vi "PicoScope4000aAdvancedTriggerSettings.vi"(0 "handle in":i16, 5 "error in":errorcluster, 6 "Trigger Conditions":T4 {"Channel H" items=["Don't Care", "True", "False"]; "Channel G" items=["Don't Care", "True", "False"]; "Channel F" items=["Don't Care", "True", "False"]; "Channel E" items=["Don't Care", "True", "False"]; "PWQ" items=["Don't Care", "True", "False"]; "Aux" items=["Don't Care", "True", "False"]; "Ext" items=["Don't Care", "True", "False"]; "Channel D" items=["Don't Care", "True", "False"]; "Channel C" items=["Don't Care", "True", "False"]; "Channel B" items=["Don't Care", "True", "False"]; "Channel A" items=["Don't Care", "True", "False"]; "Condition Logic" items=["AND", "OR", "XOR"]}, 8 "Channel Trigger Properties":T2 {"Channel H Trigger Properties"."Direction" items=["Above / Inside", "Below / Outside", "Rising / Enter", "Falling / Exit", "Rising or Falling / Enter or Exit", "Above Lower", "Below Lower", "Rising Lower", "Falling Lower", "Positive Runt", "Negative Runt"]; "Channel H Trigger Properties"."Threshold Mode" items=["Level", "Window"]; "Channel G Trigger Properties"."Direction" items=["Above / Inside", "Below / Outside", "Rising / Enter", "Falling / Exit", "Rising or Falling / Enter or Exit", "Above Lower", "Below Lower", "Rising Lower", "Falling Lower", "Positive Runt", "Negative Runt"]; "Channel G Trigger Properties"."Threshold Mode" items=["Level", "Window"]; "Channel F Trigger Properties"."Direction" items=["Above / Inside", "Below / Outside", "Rising / Enter", "Falling / Exit", "Rising or Falling / Enter or Exit", "Above Lower", "Below Lower", "Rising Lower", "Falling Lower", "Positive Runt", "Negative Runt"]; "Channel F Trigger Properties"."Threshold Mode" items=["Level", "Window"]; "Channel E Trigger Properties"."Direction" items=["Above / Inside", "Below / Outside", "Rising / Enter", "Falling / Exit", "Rising or Falling / Enter or Exit", "Above Lower", "Below Lower", "Rising Lower", "Falling Lower", "Positive Runt", "Negative Runt"]; "Channel E Trigger Properties"."Threshold Mode" items=["Level", "Window"]; "Channel D Trigger Properties"."Direction" items=["Above / Inside", "Below / Outside", "Rising / Enter", "Falling / Exit", "Rising or Falling / Enter or Exit", "Above Lower", "Below Lower", "Rising Lower", "Falling Lower", "Positive Runt", "Negative Runt"]; "Channel D Trigger Properties"."Threshold Mode" items=["Level", "Window"]; "Channel C Trigger Properties"."Direction" items=["Above / Inside", "Below / Outside", "Rising / Enter", "Falling / Exit", "Rising or Falling / Enter or Exit", "Above Lower", "Below Lower", "Rising Lower", "Falling Lower", "Positive Runt", "Negative Runt"]; "Channel C Trigger Properties"."Threshold Mode" items=["Level", "Window"]; "Channel B Trigger Properties"."Direction" items=["Above / Inside", "Below / Outside", "Rising / Enter", "Falling / Exit", "Rising or Falling / Enter or Exit", "Above Lower", "Below Lower", "Rising Lower", "Falling Lower", "Positive Runt", "Negative Runt"]; "Channel B Trigger Properties"."Threshold Mode" items=["Level", "Window"]; "Channel A Trigger Properties"."Direction" items=["Above / Inside", "Below / Outside", "Rising / Enter", "Falling / Exit", "Rising or Falling / Enter or Exit", "Above Lower", "Below Lower", "Rising Lower", "Falling Lower", "Positive Runt", "Negative Runt"]; "Channel A Trigger Properties"."Threshold Mode" items=["Level", "Window"]}, 9 "Addition Trigger Properties":T3 {"Aux. Trigger Properties (DO NOT USE)"."Direction" items=["Above / Inside", "Below / Outside", "Rising / Enter", "Falling / Exit", "Rising or Falling / Enter or Exit", "Above Lower", "Below Lower", "Rising Lower", "Falling Lower", "Positive Runt", "Negative Runt"]; "Aux. Trigger Properties (DO NOT USE)"."Threshold Mode" items=["Level", "Window"]; "Ext. Trigger Properties"."Direction" items=["Above / Inside", "Below / Outside", "Rising / Enter", "Falling / Exit", "Rising or Falling / Enter or Exit", "Above Lower", "Below Lower", "Rising Lower", "Falling Lower", "Positive Runt", "Negative Runt"]; "Ext. Trigger Properties"."Threshold Mode" items=["Level", "Window"]}, 10 "Auto Trigger (ms)":i32, 11 "Pulse Width Qualifier Conditions":T1 {"Channel H" items=["Don't Care", "True", "False"]; "Channel G" items=["Don't Care", "True", "False"]; "Channel F" items=["Don't Care", "True", "False"]; "Channel E" items=["Don't Care", "True", "False"]; "Aux" items=["Don't Care", "True", "False"]; "Ext" items=["Don't Care", "True", "False"]; "Channel D" items=["Don't Care", "True", "False"]; "Channel C" items=["Don't Care", "True", "False"]; "Channel B" items=["Don't Care", "True", "False"]; "Channel A" items=["Don't Care", "True", "False"]; "Condition Logic" items=["AND", "OR", "XOR"]}, 12 "Trigger Delay":u32, 13 "Pulse Width Qualifier Settings":T5 {"Pulse Width Type" items=["None", "Less Than", "Greater Than", "In Range", "Out of Range"]; "Direction" items=["Rising", "Falling", "Rising Lower", "Above", "Below", "Rising or Falling", "Falling Lower", "Below Lower", "Above Lower"]}) -> (14 "handle out":i16, 19 "error out":errorcluster)   [LabVIEW 2009]
doc: "This VI is an interface for the advanced trigger features of the oscilloscope.\nA simple trigger can be set using PicoScopeXXXXSettings.vi, in which case it is not necessary to use this VI."
uses:
  Program Files/Pico Technology/SDK/lib/ps4000a.dll
panel:
  in  "PWQ Info Action XOR":bool
  in  "PWQ Info Action OR":bool
  in  "SetTrigger Info Action XOR":bool
  out "XOR Debug Array":u32[][](array[numeric])
  in  "SetTrigger Info Action OR":bool
  # "For Condition Logic Suggested settings;\nFor AND, XOR logic-(parallel triggers)\nUse level-type triggers (Level or Inside/outside Window Triggers)\n\nFor OR logic- (single channel)\nUse edge types (e.g. rising, falling, entering window)"
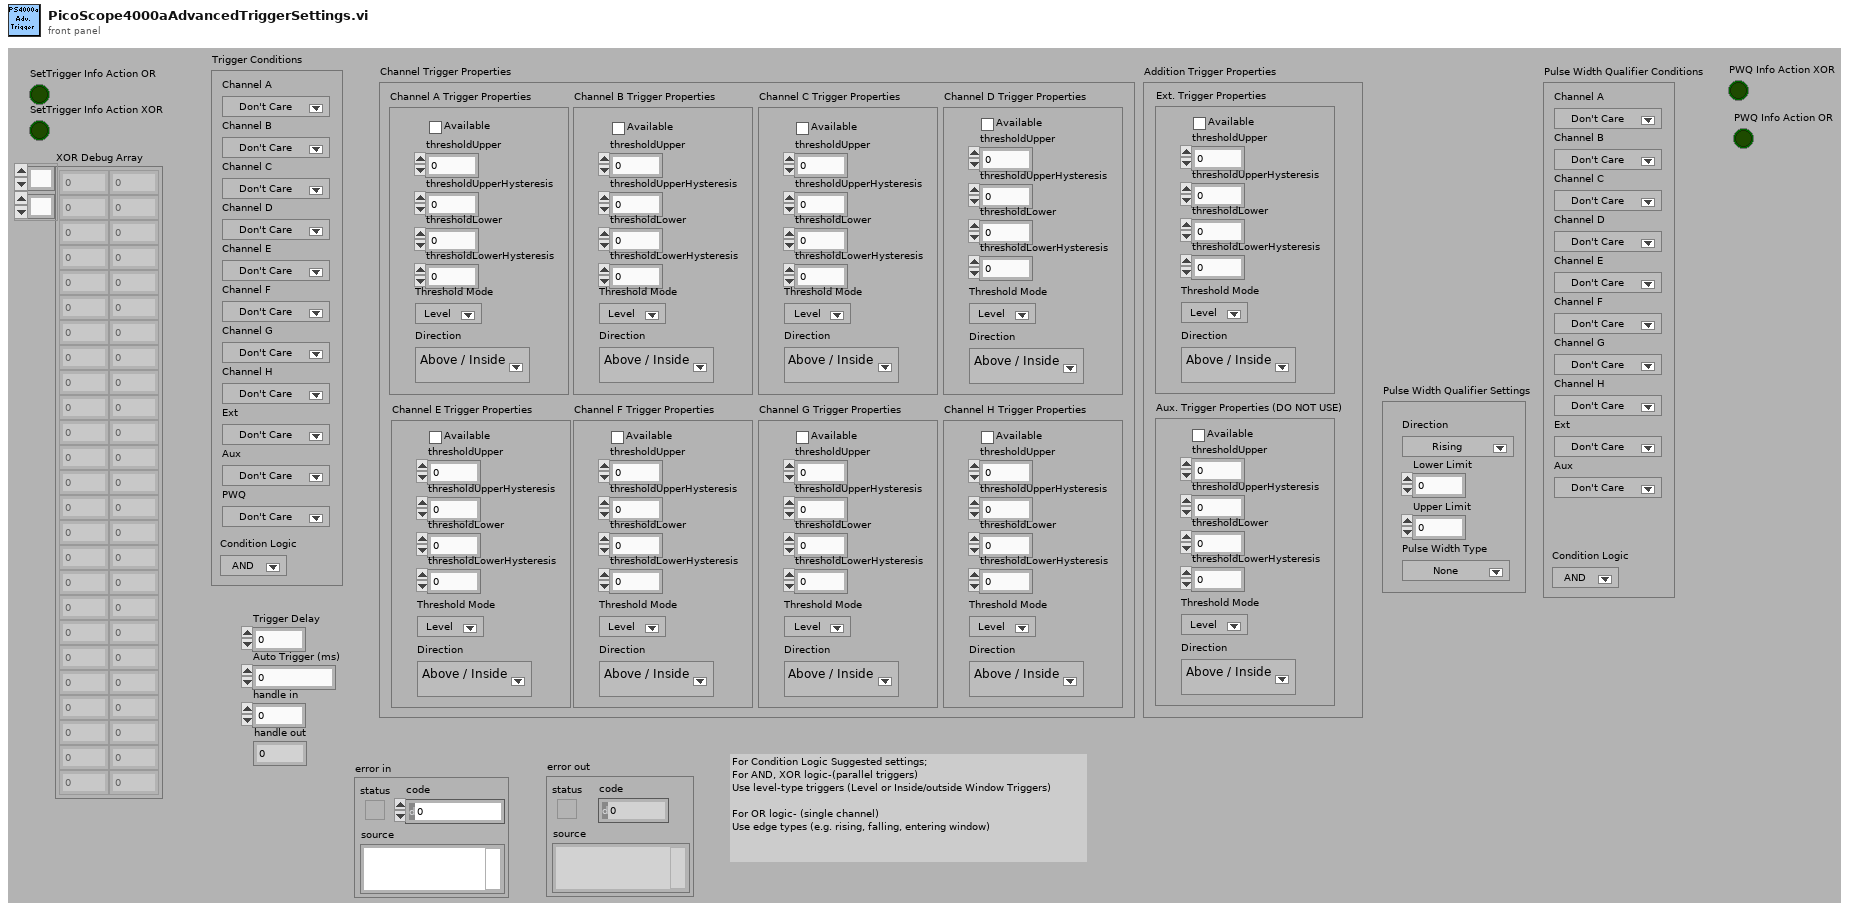
[diagram p1: front panel]
types:
  T1 = cluster{"Channel A":u16, "Channel B":u16, "Channel C":u16, "Channel D":u16, "Channel E":u16, "Channel F":u16, "Channel G":u16, "Channel H":u16, "Ext":u16, "Aux":u16, "Condition Logic":u16}
  T2 = cluster{"Channel A Trigger Properties":cluster{"thresholdUpper":i16, "thresholdUpperHysteresis":u16, "thresholdLower":i16, "thresholdLowerHysteresis":u16, "Threshold Mode":i32, "Direction":i32, "Available":bool}, "Channel B Trigger Properties":cluster{"thresholdUpper":i16, "thresholdUpperHysteresis":u16, "thresholdLower":i16, "thresholdLowerHysteresis":u16, "Threshold Mode":i32, "Direction":i32, "Available":bool}, "Channel C Trigger Properties":cluster{"thresholdUpper":i16, "thresholdUpperHysteresis":u16, "thresholdLower":i16, "thresholdLowerHysteresis":u16, "Threshold Mode":i32, "Direction":i32, "Available":bool}, "Channel D Trigger Properties":cluster{"thresholdUpper":i16, "thresholdUpperHysteresis":u16, "thresholdLower":i16, "thresholdLowerHysteresis":u16, "Threshold Mode":i32, "Direction":i32, "Available":bool}, "Channel E Trigger Properties":cluster{"thresholdUpper":i16, "thresholdUpperHysteresis":u16, "thresholdLower":i16, "thresholdLowerHysteresis":u16, "Threshold Mode":i32, "Direction":i32, "Available":bool}, "Channel F Trigger Properties":cluster{"thresholdUpper":i16, "thresholdUpperHysteresis":u16, "thresholdLower":i16, "thresholdLowerHysteresis":u16, "Threshold Mode":i32, "Direction":i32, "Available":bool}, "Channel G Trigger Properties":cluster{"thresholdUpper":i16, "thresholdUpperHysteresis":u16, "thresholdLower":i16, "thresholdLowerHysteresis":u16, "Threshold Mode":i32, "Direction":i32, "Available":bool}, "Channel H Trigger Properties":cluster{"thresholdUpper":i16, "thresholdUpperHysteresis":u16, "thresholdLower":i16, "thresholdLowerHysteresis":u16, "Threshold Mode":i32, "Direction":i32, "Available":bool}}
  T3 = cluster{"Ext. Trigger Properties":cluster{"thresholdUpper":i16, "thresholdUpperHysteresis":u16, "thresholdLower":i16, "thresholdLowerHysteresis":u16, "Threshold Mode":i32, "Direction":i32, "Available":bool}, "Aux. Trigger Properties (DO NOT USE)":cluster{"thresholdUpper":i16, "thresholdUpperHysteresis":u16, "thresholdLower":i16, "thresholdLowerHysteresis":u16, "Threshold Mode":i32, "Direction":i32, "Available":bool}}
  T4 = cluster{"Channel A":u16, "Channel B":u16, "Channel C":u16, "Channel D":u16, "Channel E":u16, "Channel F":u16, "Channel G":u16, "Channel H":u16, "Ext":u16, "Aux":u16, "PWQ":u16, "Condition Logic":u16}
  T5 = cluster{"Direction":u32, "Lower Limit":u32, "Upper Limit":u32, "Pulse Width Type":u32}
  T6 = cluster{"status":bool, "code":u32, "source":string}
  T7 = cluster{"status":bool, "code":u32, "source":string}[]
  T8 = cluster{"thresholdUpper":i16, "thresholdUpperHysteresis":u16, "thresholdLower":i16, "thresholdLowerHysteresis":u16, "Threshold Mode":i32, "Direction":i32, "Available":bool}[]
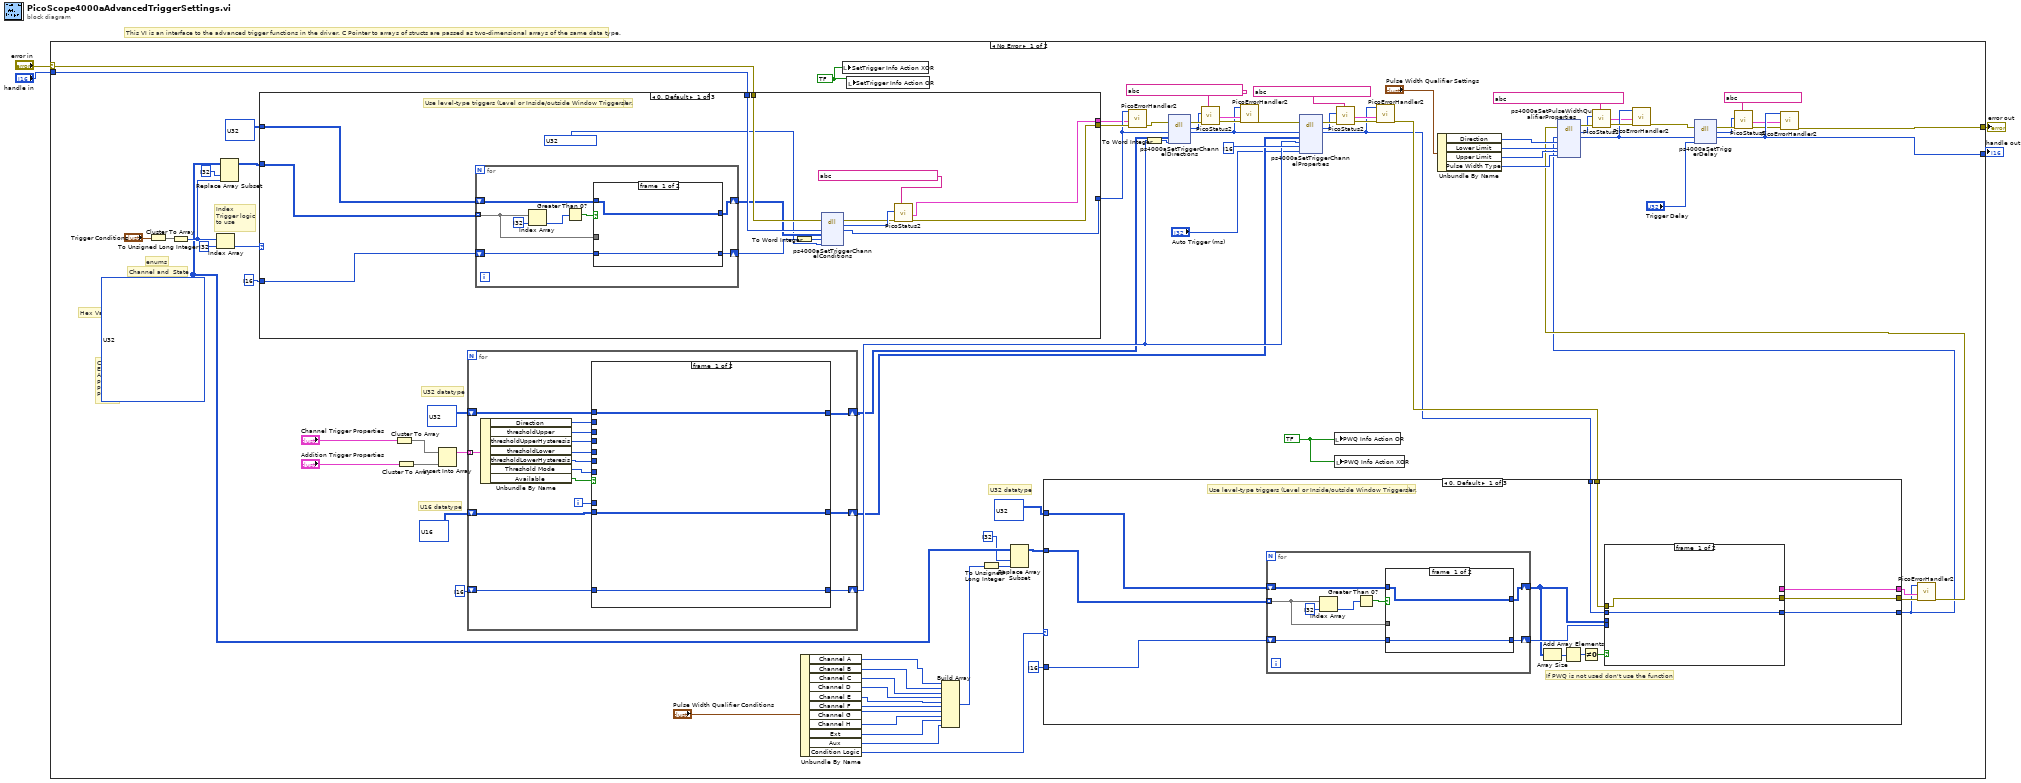
[diagram p0: block diagram]
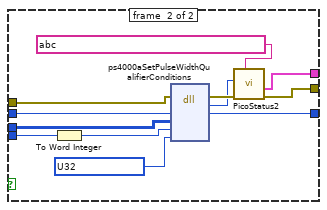
[diagram p2: hidden frame]
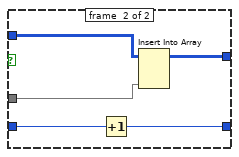
[diagram p3: hidden frame]
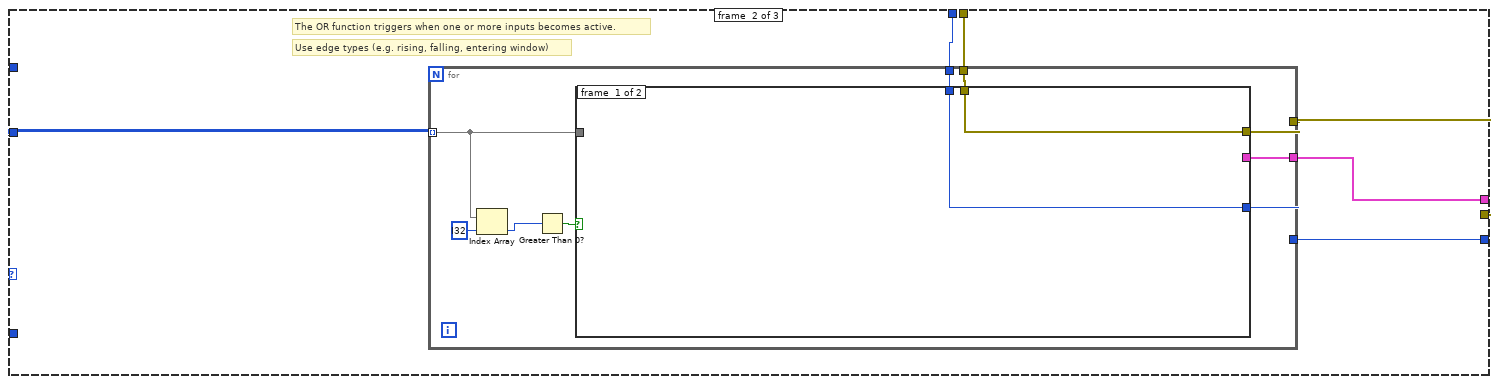
[diagram p4: hidden frame]
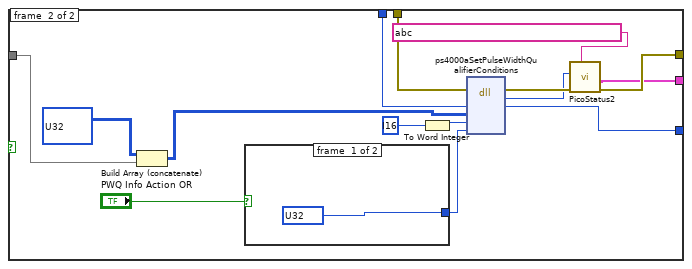
[diagram p5: hidden frame]
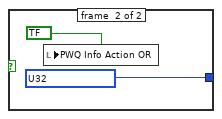
[diagram p6: hidden frame]
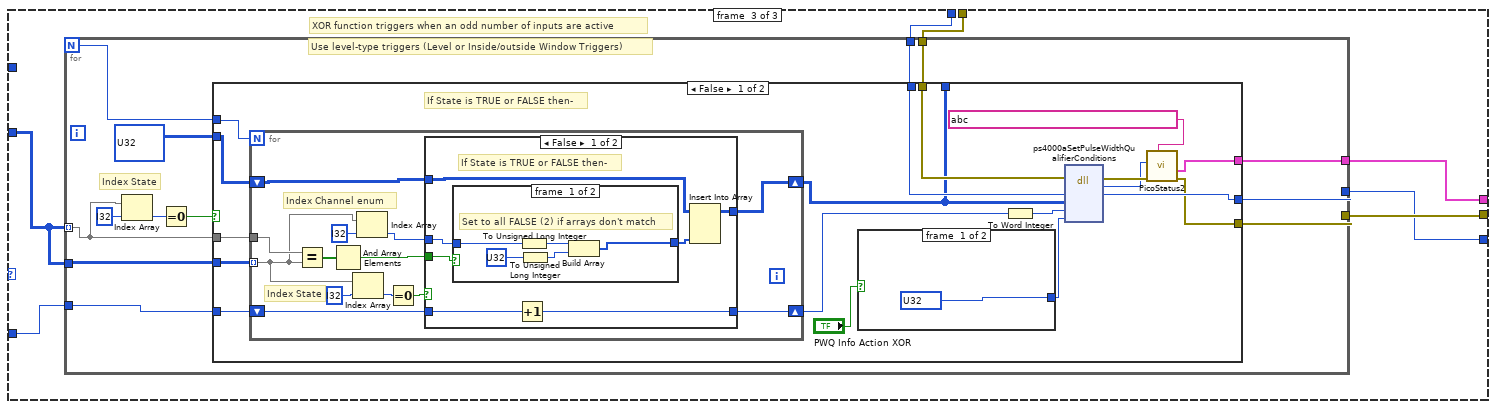
[diagram p7: hidden frame]
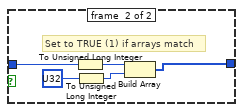
[diagram p8: hidden frame]
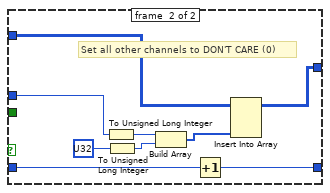
[diagram p9: hidden frame]
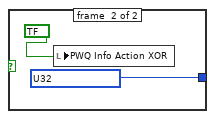
[diagram p10: hidden frame]
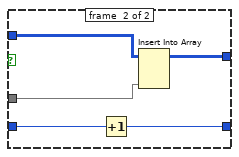
[diagram p12: hidden frame]
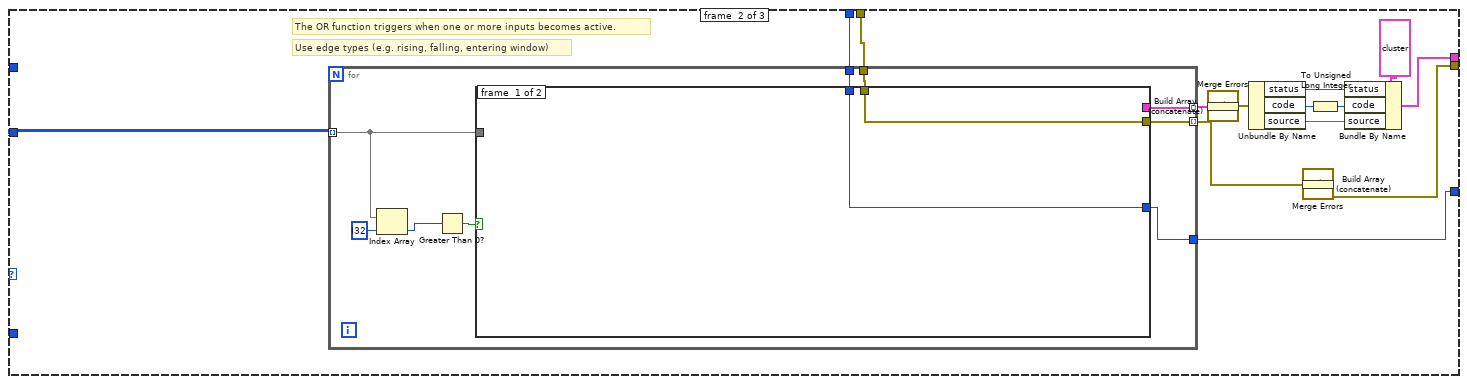
[diagram p13: hidden frame]
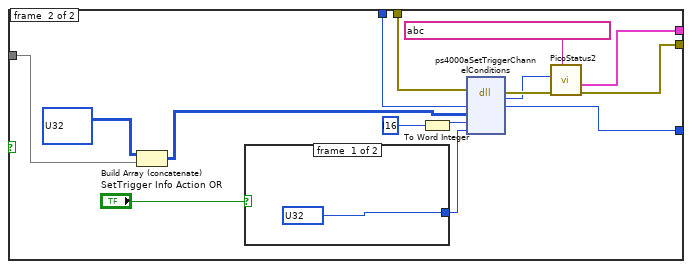
[diagram p14: hidden frame]
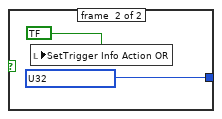
[diagram p15: hidden frame]
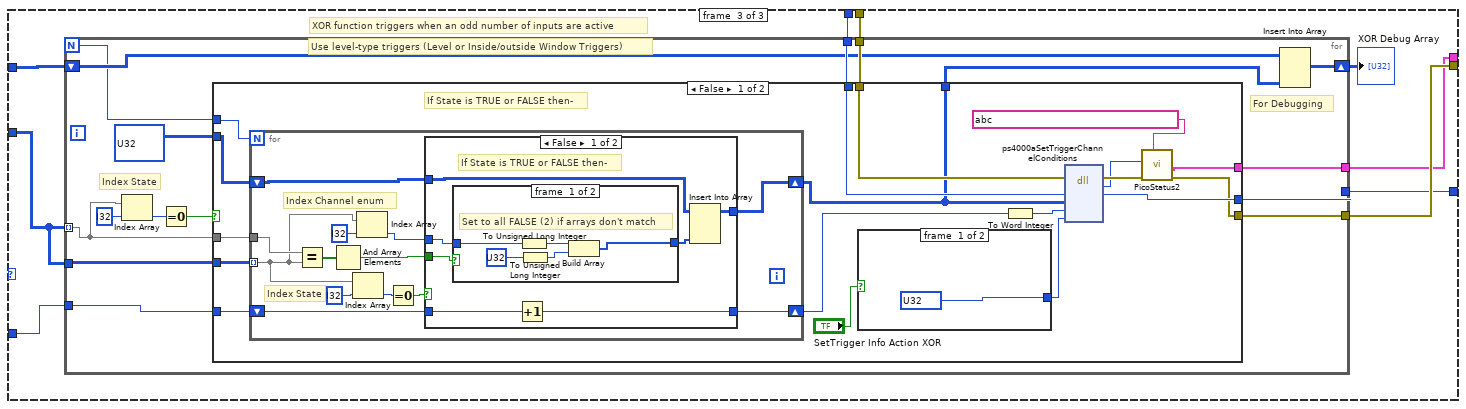
[diagram p16: hidden frame]
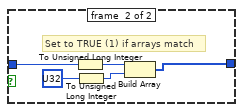
[diagram p17: hidden frame]
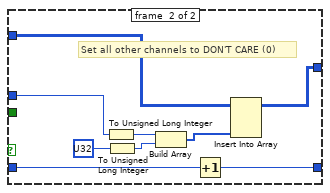
[diagram p18: hidden frame]
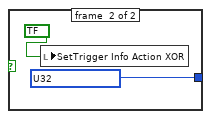
[diagram p19: hidden frame]
diagram:
  # "This VI is an interface to the advanced trigger functions in the driver. C Pointer to arrays of structs are passed as two-dimensional arrays of the same data type."
  n1 = case shown="No Error" "error in" {
    selector: "error in" -> [w59 w459]
    tunnel: "handle in" -> [w58 w460]
    tunnel: [w74 w460] -> w2
    tunnel: [w75 w459] -> w1
    frame #0 {
      w33 = bool ? ("PWQ Info Action XOR")
      w65 = bool ? ("Boolean")
      w48 = u32[][] ?
      # "U32 datatype"
      # "Index\nTrigger logic\nto use"
      # "enums"
      # "Ch H\nExt\nAux\nPWQ\nPort0\nPort1"
      # "Channel and  State"
      # "Hex Values"
      # "U16 datatype"
      # "U32 datatype"
      n2 = Cluster To Array(cluster="Trigger Conditions") -> (array=w82:u16[])
      n3 = To Unsigned Long Integer(number=w82) -> (unsigned 32bit integer=w77:u32[])
      n4 = Index Array(array=w77, index=i32 ?) -> (element=w64:u32)
      n5 = Replace Array Subset(array=w48, new element=w77, index (col)=i32 ? ("disabled index (col)")) -> (w63:u32[][])  [unwired: 1 in]
      n6 = case shown="0, Default" w64 {
        tunnel: u32[][] ? -> [w267 _ w332]
        tunnel: i16 ? -> [w266 _ w329]
        tunnel: w59 -> [w263 w298 w336]
        tunnel: w58 -> [w262 w297 w335]
        tunnel: [w253 w293 w334] -> w61
        tunnel: [w259 w296 w333] -> w60
        tunnel: w63 -> [w258 w295 w330]
        tunnel: [w254 w287 w328] -> w9
        frame #0 {
          w260 = u32 ? items=["CLEAR + ADD", "CLEAR", "ADD"] ("Condition Action")
          # "AND function requires both inputs to be active before it will trigger."
          # "Use level-type triggers (Level or Inside/outside Window Triggers)"
          n7 = for {
            shift-right: [w274] -> w264
            shift-left: w266 -> [w273]
            shift-right: [w272] -> w261
            shift-left: w267 -> [w275]
            tunnel: w258 -> [w270] mode=indexing
            n8 = Index Array(array=w270, index=i32 ?) -> (element=w269:u32)
            n9 = Greater Than 0?(x=w269) -> (x > 0?=w271:bool)
            n10 = case shown="True" w271 {
              tunnel: w275 -> [w277 w282]
              tunnel: [w277 w281] -> w272
              tunnel: [w276 w280] -> w274
              tunnel: w273 -> [w276 w279]
              tunnel: w270 -> [_ w278]
              frame #0 {
              }
              frame #1 {
                n11 = Increment(x=w279) -> (x+1=w280:i16)
                n12 = Insert Into Array(array=w282, new element=w278) -> (w281:u32[][])  [unwired: 2 in]
              }
            }
          }
          n13 = To Word Integer(number=w264) -> (16bit integer=w265:i16)
          n14 = dll-call lib="/Program Files/Pico Technology/SDK/lib/ps4000a.dll" fn="ps4000aSetTriggerChannelConditions" ("ps3000.dll:_ps3000_open_unit@0")(error in=w263, "handle"=w262, "conditions"=w261, "nConditions"=w265, "info"=w260) -> (error out=w255:errorcluster, "PICO_STATUS"=w256:u32, "handle"=w259:i16)  [unwired: 5 in, 1 out]
          n15 = call "PicoStatus2.vi"("PICO source"=string ? ("source"), "Error in"=w255, "PICO STATUS"=w256) -> ("error out"=w253:errorcluster, "PICO_STATUS out"=w254:T6)  [unwired: 5 in]
        }
        frame #1 {
          # "Use edge types (e.g. rising, falling, entering window)"
          # "The OR function triggers when one or more inputs becomes active."
          n16 = for {
            tunnel: w298 -> [w307]
            tunnel: w297 -> [w306]
            tunnel: [w305] -> w294 mode=indexing
            tunnel: [w304] -> w296
            tunnel: w295 -> [w302] mode=indexing
            tunnel: [w299] -> w286 mode=indexing
            n17 = Index Array(array=w302, index=i32 ?) -> (element=w301:u32)
            n18 = Greater Than 0?(x=w301) -> (x > 0?=w300:bool)
            n19 = case shown="True" w300 {
              tunnel: w307 -> [w308 w323]
              tunnel: w306 -> [w309 w322]
              tunnel: [w308 w312] -> w305
              tunnel: [w309 w320] -> w304
              tunnel: w302 -> [_ w315]
              tunnel: [_ w310] -> w299
              frame #0 {
              }
              frame #1 {
                n20 = Build Array (concatenate)(u32[][] ?, w315) -> (w317:u32[][])
                n21 = case shown="True" "SetTrigger Info Action OR" {
                  tunnel: [w325 w327] -> w321
                  frame #0 {
                    w325 = u32 ? items=["CLEAR", "ADD", "CLEAR + ADD"] ("Condition Action")
                  }
                  frame #1 {
                    w327 = u32 ? items=["CLEAR", "ADD", "CLEAR + ADD"] ("Condition Action")
                    n22 = local write "SetTrigger Info Action OR"(bool ? ("Boolean")) -> ()
                  }
                }
                n23 = To Word Integer(number=i16 ?) -> (16bit integer=w324:i16)
                n24 = dll-call lib="/Program Files/Pico Technology/SDK/lib/ps4000a.dll" fn="ps4000aSetTriggerChannelConditions" ("ps3000.dll:_ps3000_open_unit@0")(error in=w323, "handle"=w322, "conditions"=w317, "nConditions"=w324, "info"=w321) -> (error out=w314:errorcluster, "PICO_STATUS"=w311:u32, "handle"=w320:i16)  [unwired: 5 in, 1 out]
                n25 = call "PicoStatus2.vi"("PICO source"=string ? ("source"), "Error in"=w314, "PICO STATUS"=w311) -> ("error out"=w312:errorcluster, "PICO_STATUS out"=w310:T6)  [unwired: 5 in]
              }
            }
          }
          n26 = Build Array (concatenate)(w286) -> (w284:T7)
          n27 = call <vilib>:"Merge Errors.vi"("error array in"=w284) -> ("error out"=w285:errorcluster)  [unwired: 6 in]
          n28 = Unbundle By Name(w285) -> ("status"=w289:bool, "code"=w292:i32, "source"=w290:string)
          n29 = Build Array (concatenate)(w294) -> (w283:errorcluster[])
          n30 = call <vilib>:"Merge Errors.vi"("error array in"=w283) -> ("error out"=w293:errorcluster)  [unwired: 6 in]
          n31 = To Unsigned Long Integer(number=w292) -> (unsigned 32bit integer=w291:u32)
          n32 = Bundle By Name(cluster=T6 ? ("PICO_STATUS in"), "status"=w289, "code"=w291, "source"=w290) -> (w287:T6)
        }
        frame #2 {
          # "Use level-type triggers (Level or Inside/outside Window Triggers)"
          # "XOR function triggers when an odd number of inputs are active"
          n33 = for {
            N -> [w345]
            tunnel: w336 -> [w352]
            tunnel: w335 -> [w351]
            tunnel: [w350] -> w334
            tunnel: [w349] -> w333
            shift-right: [w347] -> w331
            shift-left: w332 -> [w348]
            tunnel: w330 -> [w339] mode=indexing
            tunnel: w330 -> [w342]
            tunnel: w329 -> [w343]
            tunnel: [w337] -> w328
            # "Index State"
            # "For Debugging"
            n34 = Index Array(array=w339, index=i32 ?) -> (element=w340:u32)
            n35 = Equal To 0?(x=w340) -> (x = 0?=w338:bool)
            n36 = case shown="False" w338 {
              tunnel: w352 -> [w370 w413]
              tunnel: w351 -> [w369 w414]
              tunnel: [w354 w413] -> w350
              tunnel: [w368 w414] -> w349
              tunnel: [w366 w415] -> w346
              tunnel: w345 -> [w365 _]
              tunnel: u32[][] ? -> [w364 w415]
              tunnel: w343 -> [w363 _]
              tunnel: w342 -> [w362 _]
              tunnel: w339 -> [w361 _]
              tunnel: [w353 _] -> w337
              frame #0 {
                # "If State is TRUE or FALSE then-"
                n37 = for {
                  N: w365 -> [_]
                  shift-right: [w382] -> w367
                  shift-left: w363 -> [w383]
                  shift-right: [w371] -> w366
                  shift-left: w364 -> [w372]
                  tunnel: w361 -> [w379]
                  tunnel: w362 -> [w375] mode=indexing
                  # "Index State"
                  # "Index Channel enum"
                  n38 = Equal?(x=w379, y=w375) -> (x = y?=w373:bool[])
                  n39 = And Array Elements(Boolean array=w373) -> (logical AND=w378:bool)
                  n40 = Index Array(array=w375, index=i32 ?) -> (element=w376:u32)
                  n41 = Index Array(array=w375, index=i32 ?) -> (element=w380:u32)
                  n42 = Equal To 0?(x=w376) -> (x = 0?=w374:bool)
                  n43 = case shown="False" w374 {
                    tunnel: w383 -> [w390 w401]
                    tunnel: [w389 w402] -> w382
                    tunnel: w380 -> [w388 w405]
                    tunnel: w378 -> [w387 _]
                    tunnel: w372 -> [w386 w404]
                    tunnel: [w384 w403] -> w371
                    frame #0 {
                      # "If State is TRUE or FALSE then-"
                      n44 = case shown="True" w387 {
                        tunnel: [w395 w400] -> w385
                        tunnel: w388 -> [w394 w399]
                        frame #0 {
                          # "Set to all FALSE (2) if arrays don't match"
                          n45 = To Unsigned Long Integer(number=w394) -> (unsigned 32bit integer=w392:u32)
                          n46 = To Unsigned Long Integer(number=u32 ?) -> (unsigned 32bit integer=w393:u32)
                          n47 = Build Array(w392, w393) -> (w395:u32[])
                        }
                        frame #1 {
                          # "Set to TRUE (1) if arrays match"
                          n48 = To Unsigned Long Integer(number=w399) -> (unsigned 32bit integer=w397:u32)
                          n49 = To Unsigned Long Integer(number=u32 ?) -> (unsigned 32bit integer=w398:u32)
                          n50 = Build Array(w397, w398) -> (w400:u32[])
                        }
                      }
                      n51 = Increment(x=w390) -> (x+1=w389:i16)
                      n52 = Insert Into Array(array=w386, new element=w385) -> (w384:u32[][])  [unwired: 2 in]
                    }
                    frame #1 {
                      # "Set all other channels to DON'T CARE (0)"
                      n53 = To Unsigned Long Integer(number=w405) -> (unsigned 32bit integer=w407:u32)
                      n54 = To Unsigned Long Integer(number=u32 ?) -> (unsigned 32bit integer=w408:u32)
                      n55 = Build Array(w407, w408) -> (w409:u32[])
                      n56 = Increment(x=w401) -> (x+1=w402:i16)
                      n57 = Insert Into Array(array=w404, new element=w409) -> (w403:u32[][])  [unwired: 2 in]
                    }
                  }
                }
                n58 = case shown="True" "SetTrigger Info Action XOR" {
                  tunnel: [w410 w412] -> w358
                  frame #0 {
                    w410 = u32 ? items=["CLEAR + ADD", "CLEAR", "ADD"] ("Condition Action")
                  }
                  frame #1 {
                    w412 = u32 ? items=["CLEAR + ADD", "CLEAR", "ADD"] ("Condition Action")
                    n59 = local write "SetTrigger Info Action XOR"(bool ? ("Boolean")) -> ()
                  }
                }
                n60 = To Word Integer(number=w367) -> (16bit integer=w360:i16)
                n61 = dll-call lib="/Program Files/Pico Technology/SDK/lib/ps4000a.dll" fn="ps4000aSetTriggerChannelConditions" ("ps3000.dll:_ps3000_open_unit@0")(error in=w370, "handle"=w369, "conditions"=w366, "nConditions"=w360, "info"=w358) -> (error out=w357:errorcluster, "PICO_STATUS"=w356:u32, "handle"=w368:i16)  [unwired: 5 in, 1 out]
                n62 = call "PicoStatus2.vi"("PICO source"=string ? ("source"), "Error in"=w357, "PICO STATUS"=w356) -> ("error out"=w354:errorcluster, "PICO_STATUS out"=w353:T6)  [unwired: 5 in]
              }
              frame #1 {
              }
            }
            n63 = Insert Into Array(array=w348, new element=w346) -> (w347:u32[][])  [unwired: 2 in]
          }
          "XOR Debug Array" <- w331
        }
      }
      n64 = Cluster To Array(cluster="Channel Trigger Properties") -> (array=w54:T8)
      n65 = Cluster To Array(cluster="Addition Trigger Properties") -> (array=w52:T8)
      n66 = Insert Into Array(array=w54, new element=w52) -> (w53:T8)  [unwired: 1 in]
      n67 = for {
        tunnel: w53 -> [w416] mode=indexing
        shift-right: [w423] -> w85
        shift-left: i16 ? -> [w422]
        shift-right: [w420] -> w79
        shift-left: u16[][] ? -> [w421]
        shift-right: [w419] -> w80
        shift-left: u32[][] ? -> [w418]
        i -> [w424]
        n68 = Unbundle By Name(w416) -> ("Direction"=w417:i32, "thresholdUpper"=w430:i16, "thresholdUpperHysteresis"=w429:u16, "thresholdLower"=w428:i16, "thresholdLowerHysteresis"=w427:u16, "Threshold Mode"=w426:i32, "Available"=w425:bool)
        n69 = case shown="True" w425 {
          tunnel: w430 -> [_ w458]
          tunnel: w429 -> [_ w440]
          tunnel: w428 -> [_ w439]
          tunnel: w427 -> [_ w438]
          tunnel: w426 -> [_ w434]
          tunnel: w424 -> [_ w448]
          tunnel: [w433 w456] -> w423
          tunnel: w422 -> [w433 w455]
          tunnel: [w432 w453] -> w420
          tunnel: w421 -> [w432 w452]
          tunnel: [w431 w451] -> w419
          tunnel: w418 -> [w431 w450]
          tunnel: w417 -> [_ w447]
          frame #0 {
          }
          frame #1 {
            # "\"0\" constants for Byte stuffing for U32"
            n70 = To Unsigned Word Integer(number=w458) -> (unsigned 16bit integer=w442:u16)
            n71 = To Unsigned Word Integer(number=w440) -> (unsigned 16bit integer=w441:u16)
            n72 = To Unsigned Word Integer(number=w439) -> (unsigned 16bit integer=w437:u16)
            n73 = To Unsigned Word Integer(number=w438) -> (unsigned 16bit integer=w443:u16)
            n74 = To Unsigned Word Integer(number=w448) -> (unsigned 16bit integer=w444:u16)
            n75 = To Unsigned Word Integer(number=w434) -> (unsigned 16bit integer=w435:u16)
            n76 = To Unsigned Long Integer(number=w447) -> (unsigned 32bit integer=w446:u32)
            n77 = To Unsigned Long Integer(number=w448) -> (unsigned 32bit integer=w445:u32)
            n78 = Build Array(w445, w446) -> (w449:u32[])
            n79 = Build Array(w442, w441, w437, w443, w444, u16 ? ("element"), w435, u16 ? ("element")) -> (w454:u16[])
            n80 = Insert Into Array(array=w450, new element=w449) -> (w451:u32[][])  [unwired: 2 in]
            n81 = Insert Into Array(array=w452, new element=w454) -> (w453:u16[][])  [unwired: 2 in]
            n82 = Increment(x=w455) -> (x+1=w456:i16)
          }
        }
      }
      n83 = Unbundle By Name("Pulse Width Qualifier Conditions") -> ("Channel A"=w43:u16, "Channel B"=w42:u16, "Channel C"=w41:u16, "Channel D"=w40:u16, "Channel E"=w39:u16, "Channel F"=w38:u16, "Channel G"=w37:u16, "Channel H"=w36:u16, "Ext"=w35:u16, "Aux"=w34:u16, "Condition Logic"=w51:u16)
      n84 = local write "SetTrigger Info Action XOR"(w65) -> ()
      n85 = local write "SetTrigger Info Action OR"(w65) -> ()
      n86 = Build Array(w43, w42, w41, w40, w39, w38, w37, w36, w35, w34) -> (w78:u16[])
      n87 = To Unsigned Long Integer(number=w78) -> (unsigned 32bit integer=w47:u32[])
      n88 = Replace Array Subset(array=w48, new element=w47, index (col)=i32 ? ("disabled index (col)")) -> (w46:u32[][])  [unwired: 1 in]
      n89 = call "PicoErrorHandler2.vi"("error in (no error)"=w61, "PICO_STATUS in"=w9, "handle In"=w60) -> ("error out"=w67:errorcluster)  [unwired: 8 in]
      n90 = To Word Integer(number=w85) -> (16bit integer=w86:i16)
      n91 = dll-call lib="/Program Files/Pico Technology/SDK/lib/ps4000a.dll" fn="ps4000aSetTriggerChannelDirections" ("ps3000.dll:_ps3000_open_unit@0")(error in=w67, "handle"=w60, "directions"=w80, "nDirections"=w86) -> (error out=w14:errorcluster, "PICO_STATUS"=w13:u32, "handle"=w12:i16)  [unwired: 4 in, 1 out]
      n92 = call "PicoStatus2.vi"("PICO source"=string ? ("source"), "Error in"=w14, "PICO STATUS"=w13) -> ("error out"=w16:errorcluster, "PICO_STATUS out"=w15:T6)  [unwired: 5 in]
      n93 = call "PicoErrorHandler2.vi"("error in (no error)"=w16, "PICO_STATUS in"=w15, "handle In"=w12) -> ("error out"=w10:errorcluster)  [unwired: 8 in]
      n94 = dll-call lib="/Program Files/Pico Technology/SDK/lib/ps4000a.dll" fn="ps4000aSetTriggerChannelProperties" ("ps3000.dll:_ps3000_open_unit@0")(error in=w10, "handle"=w12, "channelProperties"=w79, "nChannelProperties"=w85, "auxOutputEnable"=i16 ?, "autoTriggerMilliseconds"="Auto Trigger (ms)") -> (error out=w21:errorcluster, "PICO_STATUS"=w20:u32, "handle"=w17:i16)  [unwired: 6 in, 1 out]
      n95 = local write "PWQ Info Action OR"(w33) -> ()
      n96 = local write "PWQ Info Action XOR"(w33) -> ()
      n97 = call "PicoStatus2.vi"("PICO source"=string ? ("source"), "Error in"=w21, "PICO STATUS"=w20) -> ("error out"=w23:errorcluster, "PICO_STATUS out"=w22:T6)  [unwired: 5 in]
      n98 = call "PicoErrorHandler2.vi"("error in (no error)"=w23, "PICO_STATUS in"=w22, "handle In"=w17) -> ("error out"=w18:errorcluster)  [unwired: 8 in]
      n99 = case shown="0, Default" w51 {
        tunnel: u32[][] ? -> [w105 _ _]
        tunnel: i16 ? -> [w104 _ w171]
        tunnel: w18 -> [w101 w140 w176]
        tunnel: w17 -> [w100 w139 w175]
        tunnel: [w99 w138 w174] -> w8
        tunnel: [w98 w137 w173] -> w5
        tunnel: w46 -> [w102 w136 w172]
        tunnel: [w93 w135 w170] -> w6
        frame #0 {
          # "If PWQ is not used don't use the function"
          # "AND function requires both inputs to be active before it will trigger."
          # "Use level-type triggers (Level or Inside/outside Window Triggers)"
          n100 = for {
            shift-right: [w126] -> w103
            shift-left: w104 -> [w125]
            shift-right: [w124] -> w97
            shift-left: w105 -> [w127]
            tunnel: w102 -> [w122] mode=indexing
            n101 = Index Array(array=w122, index=i32 ?) -> (element=w121:u32)
            n102 = Greater Than 0?(x=w121) -> (x > 0?=w123:bool)
            n103 = case shown="True" w123 {
              tunnel: w127 -> [w129 w134]
              tunnel: [w129 w133] -> w124
              tunnel: [w128 w132] -> w126
              tunnel: w125 -> [w128 w131]
              tunnel: w122 -> [_ w130]
              frame #0 {
              }
              frame #1 {
                n104 = Increment(x=w131) -> (x+1=w132:i16)
                n105 = Insert Into Array(array=w134, new element=w130) -> (w133:u32[][])  [unwired: 2 in]
              }
            }
          }
          n106 = Array Size(array=w97) -> (size(s)=w95:i32[])
          n107 = Add Array Elements(numeric array=w95) -> (sum=w96:i32)
          n108 = Not Equal To 0?(x=w96) -> (x != 0?=w94:bool)
          n109 = case shown="True" w94 {
            tunnel: w103 -> [_ w119]
            tunnel: w101 -> [w107 w118]
            tunnel: w100 -> [w106 w117]
            tunnel: w97 -> [_ w114]
            tunnel: [w107 w109] -> w99
            tunnel: [w106 w113] -> w98
            tunnel: [_ w108] -> w93
            frame #0 {
            }
            frame #1 {
              w116 = u32 ? items=["CLEAR + ADD", "CLEAR", "ADD"] ("Condition Action")
              n110 = To Word Integer(number=w119) -> (16bit integer=w115:i16)
              n111 = dll-call lib="/Program Files/Pico Technology/SDK/lib/ps4000a.dll" fn="ps4000aSetPulseWidthQualifierConditions" ("ps3000.dll:_ps3000_open_unit@0")(error in=w118, "handle"=w117, "conditions"=w114, "nConditions"=w115, "info"=w116) -> (error out=w112:errorcluster, "PICO_STATUS"=w110:u32, "handle"=w113:i16)  [unwired: 5 in, 1 out]
              n112 = call "PicoStatus2.vi"("PICO source"=string ? ("source"), "Error in"=w112, "PICO STATUS"=w110) -> ("error out"=w109:errorcluster, "PICO_STATUS out"=w108:T6)  [unwired: 5 in]
            }
          }
        }
        frame #1 {
          # "Use edge types (e.g. rising, falling, entering window)"
          # "The OR function triggers when one or more inputs becomes active."
          n113 = for {
            tunnel: w140 -> [w149]
            tunnel: w139 -> [w148]
            tunnel: [w147] -> w138
            tunnel: [w146] -> w137
            tunnel: w136 -> [w144] mode=indexing
            tunnel: [w141] -> w135
            n114 = Index Array(array=w144, index=i32 ?) -> (element=w143:u32)
            n115 = Greater Than 0?(x=w143) -> (x > 0?=w142:bool)
            n116 = case shown="True" w142 {
              tunnel: w149 -> [w150 w165]
              tunnel: w148 -> [w151 w164]
              tunnel: [w150 w155] -> w147
              tunnel: [w151 w162] -> w146
              tunnel: w144 -> [_ w157]
              tunnel: [_ w152] -> w141
              frame #0 {
              }
              frame #1 {
                n117 = Build Array (concatenate)(u32[][] ?, w157) -> (w159:u32[][])
                n118 = case shown="True" "PWQ Info Action OR" {
                  tunnel: [w167 w169] -> w163
                  frame #0 {
                    w167 = u32 ? items=["CLEAR", "ADD", "CLEAR + ADD"] ("Condition Action")
                  }
                  frame #1 {
                    w169 = u32 ? items=["CLEAR", "ADD", "CLEAR + ADD"] ("Condition Action")
                    n119 = local write "PWQ Info Action OR"(bool ? ("Boolean")) -> ()
                  }
                }
                n120 = To Word Integer(number=i16 ?) -> (16bit integer=w166:i16)
                n121 = dll-call lib="/Program Files/Pico Technology/SDK/lib/ps4000a.dll" fn="ps4000aSetPulseWidthQualifierConditions" ("ps3000.dll:_ps3000_open_unit@0")(error in=w165, "handle"=w164, "conditions"=w159, "nConditions"=w166, "info"=w163) -> (error out=w156:errorcluster, "PICO_STATUS"=w153:u32, "handle"=w162:i16)  [unwired: 5 in, 1 out]
                n122 = call "PicoStatus2.vi"("PICO source"=string ? ("source"), "Error in"=w156, "PICO STATUS"=w153) -> ("error out"=w155:errorcluster, "PICO_STATUS out"=w152:T6)  [unwired: 5 in]
              }
            }
          }
        }
        frame #2 {
          # "Use level-type triggers (Level or Inside/outside Window Triggers)"
          # "XOR function triggers when an odd number of inputs are active"
          n123 = for {
            N -> [w185]
            tunnel: w176 -> [w189]
            tunnel: w175 -> [w188]
            tunnel: [w187] -> w174
            tunnel: [w186] -> w173
            tunnel: w172 -> [w179] mode=indexing
            tunnel: w172 -> [w182]
            tunnel: w171 -> [w183]
            tunnel: [w177] -> w170
            # "Index State"
            n124 = Index Array(array=w179, index=i32 ?) -> (element=w180:u32)
            n125 = Equal To 0?(x=w180) -> (x = 0?=w178:bool)
            n126 = case shown="False" w178 {
              tunnel: w189 -> [w207 w250]
              tunnel: w188 -> [w206 w251]
              tunnel: [w191 w250] -> w187
              tunnel: [w192 w251] -> w186
              tunnel: [w204 w252] -> _
              tunnel: w185 -> [w203 _]
              tunnel: u32[][] ? -> [w202 w252]
              tunnel: w183 -> [w201 _]
              tunnel: w182 -> [w200 _]
              tunnel: w179 -> [w199 _]
              tunnel: [w190 _] -> w177
              frame #0 {
                # "If State is TRUE or FALSE then-"
                n127 = for {
                  N: w203 -> [_]
                  shift-right: [w219] -> w205
                  shift-left: w201 -> [w220]
                  shift-right: [w208] -> w204
                  shift-left: w202 -> [w209]
                  tunnel: w199 -> [w216]
                  tunnel: w200 -> [w212] mode=indexing
                  # "Index State"
                  # "Index Channel enum"
                  n128 = Equal?(x=w216, y=w212) -> (x = y?=w210:bool[])
                  n129 = And Array Elements(Boolean array=w210) -> (logical AND=w215:bool)
                  n130 = Index Array(array=w212, index=i32 ?) -> (element=w213:u32)
                  n131 = Index Array(array=w212, index=i32 ?) -> (element=w217:u32)
                  n132 = Equal To 0?(x=w213) -> (x = 0?=w211:bool)
                  n133 = case shown="False" w211 {
                    tunnel: w220 -> [w227 w238]
                    tunnel: [w226 w239] -> w219
                    tunnel: w217 -> [w225 w242]
                    tunnel: w215 -> [w224 _]
                    tunnel: w209 -> [w223 w241]
                    tunnel: [w221 w240] -> w208
                    frame #0 {
                      # "If State is TRUE or FALSE then-"
                      n134 = case shown="True" w224 {
                        tunnel: [w232 w237] -> w222
                        tunnel: w225 -> [w231 w236]
                        frame #0 {
                          # "Set to all FALSE (2) if arrays don't match"
                          n135 = To Unsigned Long Integer(number=w231) -> (unsigned 32bit integer=w229:u32)
                          n136 = To Unsigned Long Integer(number=u32 ?) -> (unsigned 32bit integer=w230:u32)
                          n137 = Build Array(w229, w230) -> (w232:u32[])
                        }
                        frame #1 {
                          # "Set to TRUE (1) if arrays match"
                          n138 = To Unsigned Long Integer(number=w236) -> (unsigned 32bit integer=w234:u32)
                          n139 = To Unsigned Long Integer(number=u32 ?) -> (unsigned 32bit integer=w235:u32)
                          n140 = Build Array(w234, w235) -> (w237:u32[])
                        }
                      }
                      n141 = Increment(x=w227) -> (x+1=w226:i16)
                      n142 = Insert Into Array(array=w223, new element=w222) -> (w221:u32[][])  [unwired: 2 in]
                    }
                    frame #1 {
                      # "Set all other channels to DON'T CARE (0)"
                      n143 = To Unsigned Long Integer(number=w242) -> (unsigned 32bit integer=w244:u32)
                      n144 = To Unsigned Long Integer(number=u32 ?) -> (unsigned 32bit integer=w245:u32)
                      n145 = Build Array(w244, w245) -> (w246:u32[])
                      n146 = Increment(x=w238) -> (x+1=w239:i16)
                      n147 = Insert Into Array(array=w241, new element=w246) -> (w240:u32[][])  [unwired: 2 in]
                    }
                  }
                }
                n148 = case shown="True" "PWQ Info Action XOR" {
                  tunnel: [w247 w249] -> w196
                  frame #0 {
                    w247 = u32 ? items=["CLEAR + ADD", "CLEAR", "ADD"] ("Condition Action")
                  }
                  frame #1 {
                    w249 = u32 ? items=["CLEAR + ADD", "CLEAR", "ADD"] ("Condition Action")
                    n149 = local write "PWQ Info Action XOR"(bool ? ("Boolean")) -> ()
                  }
                }
                n150 = To Word Integer(number=w205) -> (16bit integer=w198:i16)
                n151 = dll-call lib="/Program Files/Pico Technology/SDK/lib/ps4000a.dll" fn="ps4000aSetPulseWidthQualifierConditions" ("ps3000.dll:_ps3000_open_unit@0")(error in=w207, "handle"=w206, "conditions"=w204, "nConditions"=w198, "info"=w196) -> (error out=w195:errorcluster, "PICO_STATUS"=w194:u32, "handle"=w192:i16)  [unwired: 5 in, 1 out]
                n152 = call "PicoStatus2.vi"("PICO source"=string ? ("source"), "Error in"=w195, "PICO STATUS"=w194) -> ("error out"=w191:errorcluster, "PICO_STATUS out"=w190:T6)  [unwired: 5 in]
              }
              frame #1 {
              }
            }
          }
        }
      }
      n153 = Unbundle By Name("Pulse Width Qualifier Settings") -> ("Direction"=w71:u32, "Lower Limit"=w70:u32, "Upper Limit"=w69:u32, "Pulse Width Type"=w68:u32)
      n154 = call "PicoErrorHandler2.vi"("error in (no error)"=w8, "PICO_STATUS in"=w6, "handle In"=w5) -> ("error out"=w7:errorcluster)  [unwired: 8 in]
      n155 = dll-call lib="/Program Files/Pico Technology/SDK/lib/ps4000a.dll" fn="ps4000aSetPulseWidthQualifierProperties" ("ps3000.dll:_ps3000_open_unit@0")(error in=w7, "handle"=w5, "direction"=w71, "lower"=w70, "upper"=w69, "type"=w68) -> (error out=w73:errorcluster, "PICO_STATUS"=w57:u32, "handle"=w25:i16)  [unwired: 6 in, 1 out]
      n156 = call "PicoStatus2.vi"("PICO source"=string ? ("source"), "Error in"=w73, "PICO STATUS"=w57) -> ("error out"=w27:errorcluster, "PICO_STATUS out"=w24:T6)  [unwired: 5 in]
      n157 = call "PicoErrorHandler2.vi"("error in (no error)"=w27, "PICO_STATUS in"=w24, "handle In"=w25) -> ("error out"=w26:errorcluster)  [unwired: 8 in]
      n158 = dll-call lib="/Program Files/Pico Technology/SDK/lib/ps4000a.dll" fn="ps4000aSetTriggerDelay" ("ps3000.dll:_ps3000_open_unit@0")(error in=w26, "handle"=w25, "delay"="Trigger Delay") -> (error out=w32:errorcluster, "PICO_STATUS"=w29:u32, "handle"=w74:i16)  [unwired: 3 in, 1 out]
      n159 = call "PicoStatus2.vi"("PICO source"=string ? ("source"), "Error in"=w32, "PICO STATUS"=w29) -> ("error out"=w31:errorcluster, "PICO_STATUS out"=w30:T6)  [unwired: 5 in]
      n160 = call "PicoErrorHandler2.vi"("error in (no error)"=w31, "PICO_STATUS in"=w30, "handle In"=w74) -> ("error out"=w75:errorcluster)  [unwired: 8 in]
    }
    frame #1 {
    }
  }
  "handle out" <- w2
  "error out" <- w1
